vi "Clear and flush table.vi"(8 "error in":errorcluster, 10 "UI GUID":string, 11 "Trace":refnum<vi>) -> (0 "error out":errorcluster)   [LabVIEW 2025, in "CAN-LIN Raw Bus Capture UI.lvlib"]
uses:
  CAN-LIN Raw Bus Capture UI.lvlib
  <vilib>/Utility/miscctls.llb/LVRowAndColumnTypeDef.ctl
  Flush Table.vi
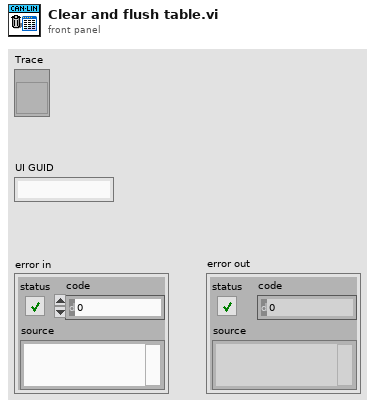
[diagram p1: front panel]
types:
  T1 = typedef "LVRowAndColumnTypeDef.ctl" = cluster{"Row":i32, "Column":i32}
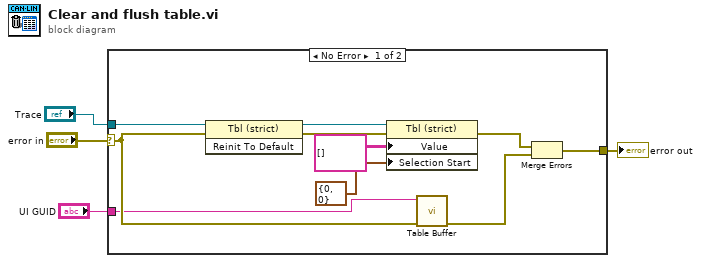
[diagram p0: block diagram]
diagram:
  n1 = case shown="No Error" "error in" {
    selector: "error in" -> [w7 w15]
    tunnel: "Trace" -> [w10 _]
    tunnel: [w6 w15] -> w2
    tunnel: "UI GUID" -> [w5 _]
    frame No Error {
      n2 = invoke class="Tbl (strict)" method="Reinit To Default"(reference=w10, error in=w7) -> (reference out=w11:refnum<vi>, error out=w12:errorcluster)  [unwired: 1 in, 1 out]
      n3 = property on="Property Node" class="Tbl (strict)"(reference=w11, error in=w12, "Value"=string[][] [], "Selection Start"=T1 {"Row"=0, "Column"=0}) -> (error out=w9:errorcluster)  [unwired: 1 out]
      n4 = call-poly "Table Buffer.vi"("error in"=w7, "UI GUID"=w5) -> ("error out"=w8:errorcluster)  [unwired: 9 in]
      n5 = Merge Errors(w9, w8) -> (w6:errorcluster)
    }
    frame Error {
    }
  }
  "error out" <- w2
